vi "Format Entry Row.vi"(7 "Project Store in":refnum<class "Project Store.lvclass">, 8 "error in":errorcluster, 10 "Now":timestamp, 11 "Time Entry":T1) -> (0 "error out":errorcluster, 3 "Row":string[](array[string]), 5 "Project Store out":refnum<class "Project Store.lvclass">)   [LabVIEW 2026]
doc: "Formats one time entry as a TimeCard listbox row, with the same seven columns in the same order as the old Update Time Entry.vi: Entry ID, Start, End, Elapsed, Project, Task, Description. Start and End are local times formatted %I:%M:%S %p. Elapsed is hh:mm:ss, rounded to whole seconds BEFORE it is split into hours, minutes and seconds, so it never shows :60. Project and Task names are looked up by ID in the Project Store; an ID it does not know is shown as the ID itself. A running entry (End Time 0) gets an empty End column and an Elapsed of Now minus Start.\n\nInputs: Time Entry; Now (used only for a running entry); Project Store in; error in.\nOutputs: Row (7 strings); Project Store out; error out.\n\nGenerated by: Claude"
uses:
  Storage/Rows/Time Entry.ctl
  Storage/Project Store/Project Store.lvclass
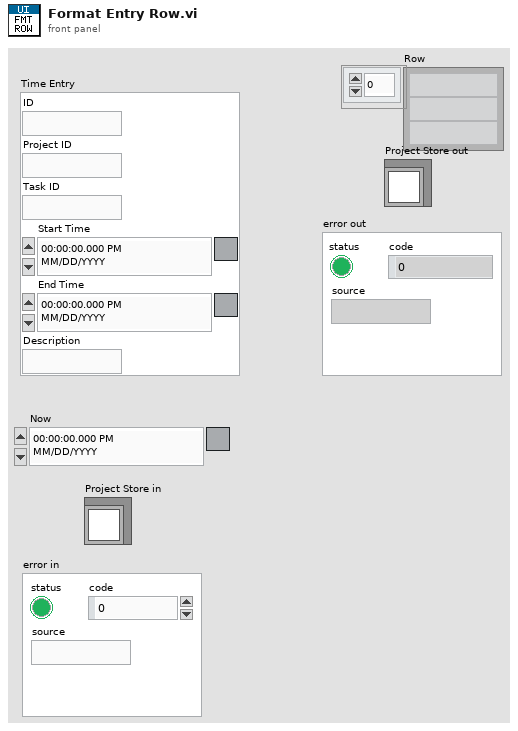
[diagram p1: front panel]
types:
  T1 = typedef "Time Entry.ctl" = cluster{"ID":string, "Project ID":string, "Task ID":string, "Start Time":timestamp, "End Time":timestamp, "Description":string}
  T2 = typedef "Project.ctl" = cluster{"ID":string, "Name":string, "Active":bool, "Sort Order":i32}
  T3 = typedef "Task.ctl" = cluster{"ID":string, "Project ID":string, "Name":string, "Active":bool, "Sort Order":i32}
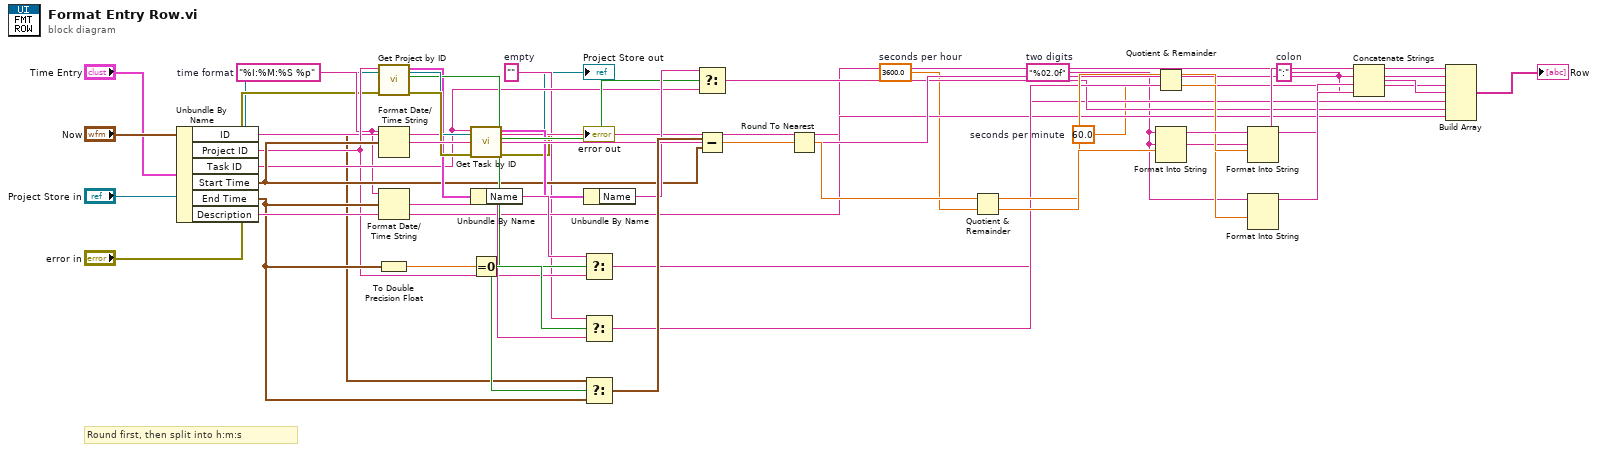
[diagram p0: block diagram]
diagram:
  w13 = 60.0  # seconds per minute
  w12 = 3600.0  # seconds per hour
  w11 = ""  # empty
  w10 = ":"  # colon
  w9 = "%02.0f"  # two digits
  w8 = "%I:%M:%S %p"  # time format
  # "Round first, then split into h:m:s"
  n1 = Unbundle By Name("Time Entry") -> ("ID"=w14:string, "Project ID"=w15:string, "Task ID"=w16:string, "Start Time"=w17:timestamp, "End Time"=w18:timestamp, "Description"=w19:string)
  n2 = call-dynamic "Get Project by ID.vi"("Project Store in"="Project Store in", "error in (no error)"="error in", "ID"=w15) -> ("error out"=w23:errorcluster, "found?"=w21:bool, "Project"=w20:T2, "Project Store out"=w22:refnum<class "Project Store.lvclass">)  [unwired: 5 in]
  n3 = Format Date/Time String(time format string (%c)=w8, seconds (now)=w17) -> (date/time string=w30:string)  [unwired: 1 out]
  n4 = Format Date/Time String(time format string (%c)=w8, seconds (now)=w18) -> (date/time string=w31:string)  [unwired: 1 out]
  n5 = To Double Precision Float(number=w18) -> (double precision float=w32:dbl)
  n6 = call-dynamic "Get Task by ID.vi"("Project Store in"=w22, "error in (no error)"=w23, "ID"=w16) -> ("error out"=→"error out":errorcluster, "found?"=w25:bool, "Task"=w24:T3, "Project Store out"=→"Project Store out":refnum<class "Project Store.lvclass">)  [unwired: 5 in]
  n7 = Unbundle By Name(w20) -> ("Name"=w26:string)
  n8 = Equal To 0?(x=w32) -> (x = 0?=w33:bool)
  n9 = Unbundle By Name(w24) -> ("Name"=w27:string)
  n10 = Select(t=w26, s=w21, f=w15) -> (s? t:f=w28:string)
  n11 = Select(t=w11, s=w33, f=w31) -> (s? t:f=w34:string)
  n12 = Select(t="Now", s=w33, f=w18) -> (s? t:f=w35:timestamp)
  n13 = Select(t=w27, s=w25, f=w16) -> (s? t:f=w29:string)
  n14 = Subtract(x=w35, y=w17) -> (x-y=w36:dbl)
  n15 = Round To Nearest(number=w36) -> (nearest integer value=w37:dbl)
  n16 = Quotient & Remainder(x=w37, y=w12) -> (x-y*floor(x/y)=w38:dbl, floor(x/y)=w39:dbl)
  n17 = Quotient & Remainder(x=w38, y=w13) -> (x-y*floor(x/y)=w40:dbl, floor(x/y)=w41:dbl)
  n18 = Format Into String(format string=w9, w39) -> (resulting string=w42:string)  [unwired: 2 in, 1 out]
  n19 = Format Into String(format string=w9, w41) -> (resulting string=w43:string)  [unwired: 2 in, 1 out]
  n20 = Format Into String(format string=w9, w40) -> (resulting string=w44:string)  [unwired: 2 in, 1 out]
  n21 = Concatenate Strings(w42, w10, w43, w10, w44) -> (w45:string)
  n22 = Build Array(w14, w30, w34, w45, w28, w29, w19) -> (→"Row":string[])
